vi "Lire_la_configuration.vi"(0 "Port COM run 1 REG":refnum<visa-resource-name>, 1 "Adresse rég":u8 caption="Adresse régulateur", 2 "error in (no error)":errorcluster caption="entrée d'erreur (pas d'erreur)") -> (3 "Programmation configuration":cluster{"Command (PV)":string, dbl}[](array[cluster]), 4 "AL haute sécu":dbl, 5 "AL basse sécu":dbl, 6 "error out":errorcluster caption="entrée d'erreur (pas d'erreur)")   [LabVIEW 2022 SP3]
uses:
  Variables globales/Variables glob EUROTHERM.vi
panel:
  out "Nom rég":string caption="Nom régulateur"
  # "lecture alarmes MODBUS"
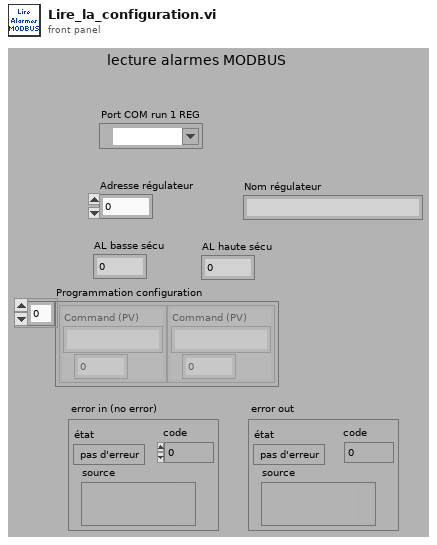
[diagram p1: front panel]
types:
  T1 = typedef "Semaphore RefNum" = refnum<k1>
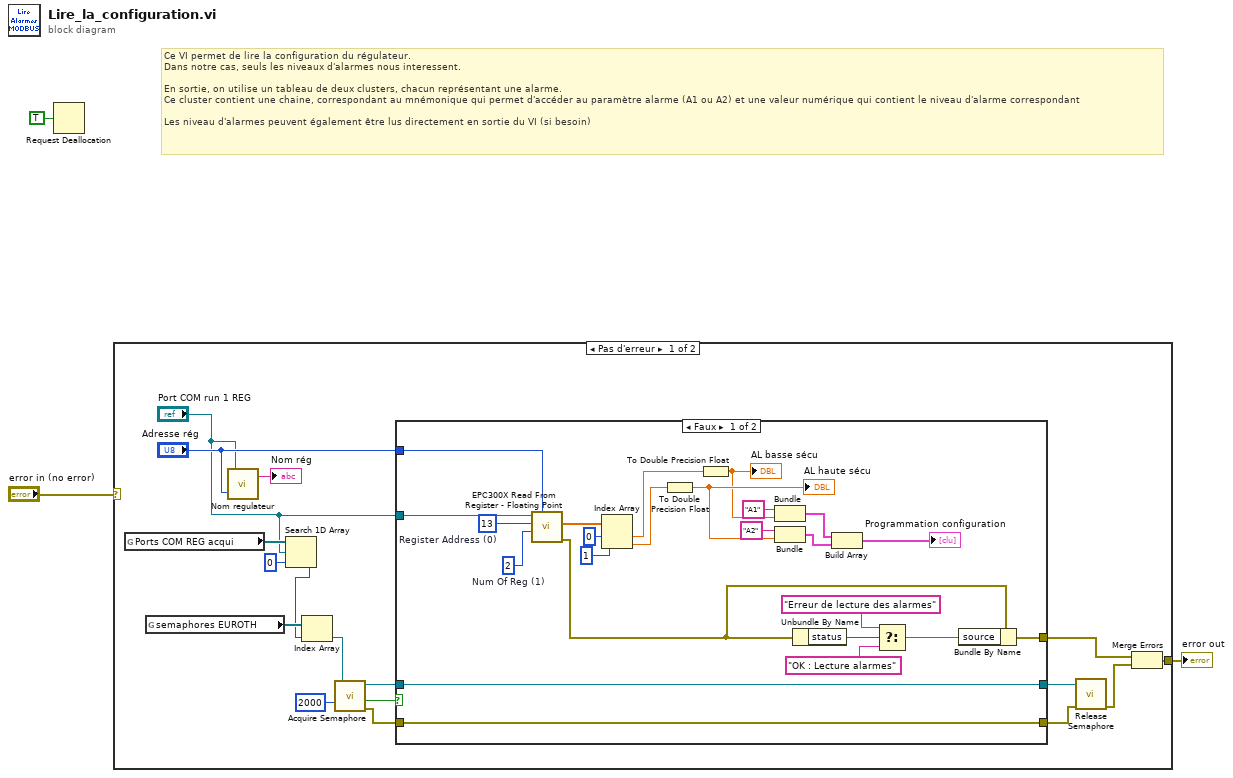
[diagram p0: block diagram]
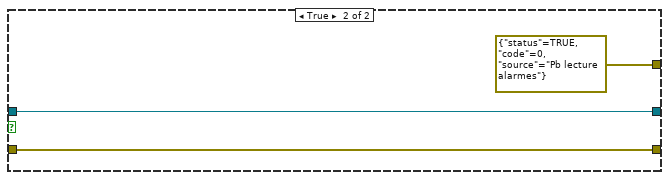
[diagram p2: hidden frame]
diagram:
  # "Ce VI permet de lire la configuration du régulateur.\nDans notre cas, seuls les niveaux d'alarmes nous interessent.\n\nEn sortie, on utilise un tableau de deux clusters, chacun représentant une alarme.\nCe cluster contient une chaine, correspondant au mnémonique qui permet d'accéder au paramètre alarme (A1 ou A2) et une valeur numérique qui contient le niveau d'alarme correspondant\n\nLes niveau d'alarmes peuvent également être lus directement en sortie du VI (si besoin)"
  n1 = Request Deallocation(TRUE ("flag")) -> ()
  n2 = case shown="Pas d'erreur" "error in (no error)" {
    selector: "error in (no error)" -> [_ w48]
    tunnel: [w12 w48] -> w2
    frame No Error {
      n3 = global read "Variables glob EUROTHERM.vi" "Ports COM REG acqui"() -> (w7:refnum<visa-resource-name>[])
      n4 = global read "Variables glob EUROTHERM.vi" "semaphores EUROTH"() -> (w11:T1[])
      n5 = call "Nom regulateur.vi"("Adresse régulateur"="Adresse rég", "Port COM run 1 REG"="Port COM run 1 REG") -> ("Nom régulateur"=→"Nom rég":string)  [unwired: 1 in]
      n6 = Search 1D Array(1D array=w7, element="Port COM run 1 REG", start index (0)=0 ("indice de départ (0)")) -> (index of element=w4:i32)
      n7 = Index Array(array=w11, index=w4) -> (element=w10:T1)
      n8 = call <vilib>:"Acquire Semaphore.vi"("ms timeout (-1)"=2000, "semaphore"=w10) -> ("error out"=w18:errorcluster, "timed out"=w20:bool, "semaphore out"=w19:T1)  [unwired: 3 in]
      n9 = case shown="Faux" w20 {
        tunnel: w19 -> [w37 w47]
        tunnel: w18 -> [w36 w46]
        tunnel: [w37 w47] -> w17
        tunnel: [w36 w46] -> w16
        tunnel: [w31 errorcluster {"status"=TRUE, "code"=0, "source"="Pb lecture alarmes"} ("error out")] -> w13
        tunnel: "Port COM run 1 REG" -> [w24 _]
        tunnel: "Adresse rég" -> [w26 _]
        frame False {
          w29 = u16 2  # Num Of Reg (1)
          w25 = u16 13  # Register Address (0)
          n10 = call "EPC300X Read From Register - Floating Point.vi"("Unit Address (1)"=w26, "Num Of Reg (1)"=w29, "Register Address (0)"=w25, "VISA session"=w24) -> ("error out"=w21:errorcluster, "Data (SGL)"=w28:sgl[])  [unwired: 2 in, 4 out]
          n11 = Index Array(array=w28, index #1=0 ("index"), index #2=1 ("indice")) -> (element #1=w23:sgl, element #2=w22:sgl)
          n12 = To Double Precision Float(number=w22) -> (double precision float=w43:dbl)
          "AL haute sécu" <- w43
          n13 = To Double Precision Float(number=w23) -> (double precision float=w42:dbl)
          "AL basse sécu" <- w42
          n14 = Bundle("Command (PV)"="A1", w42) -> (w40:cluster{"Command (PV)":string, dbl})  [unwired: 1 in]
          n15 = Bundle("Command (PV)"="A2", w43) -> (w41:cluster{"Command (PV)":string, dbl})  [unwired: 1 in]
          n16 = Unbundle By Name(w21) -> ("status"=w35:bool)
          n17 = Build Array(w40, w41) -> (→"Programmation configuration":cluster{"Command (PV)":string, dbl}[])
          n18 = Select(t="Erreur de lecture des alarmes", s=w35, f="OK : Lecture alarmes") -> (s? t:f=w32:string)
          n19 = Bundle By Name(cluster=w21, "source"=w32) -> (w31:errorcluster)
        }
        frame True {
        }
      }
      n20 = call <vilib>:"Release Semaphore.vi"("error in (no error)"=w16, "semaphore"=w17) -> ("error out"=w14:errorcluster)  [unwired: 4 in, 1 out]
      n21 = Merge Errors(w13, w14) -> (w12:errorcluster)
    }
    frame Error {
    }
  }
  "error out" <- w2
